vi "Get Input.vi"(8 "error in (no error)":errorcluster, 10 "DIO_CFG":refnum<class "DIO-Configuration.lvclass">, 11 "UI Template in":refnum<class "DIO_Panel.lvclass">) -> (0 "error out":errorcluster, 2 "Input":bool, 3 "UI Template out":refnum<class "DIO_Panel.lvclass">)   [LabVIEW 2021, in "Simulator-Channel.lvlib" / "DIO_Panel.lvlib" / "DIO_Panel.lvclass"]
uses:
  DIO_Panel.lvclass
  Dependencies/DIO-Channel.lvlibp/Channels/DIO-Channel/DIO-Configuration_class/DIO-Configuration.lvclass
  C:/Users/averna/Documents/LV Gym DEMO/Factory Pattern/Channels/Dependencies/Channel.lvlibp/Channel/Configuration_class/Configuration.lvclass
  DIO_Panel.lvclass/DIO_Panel.ctl
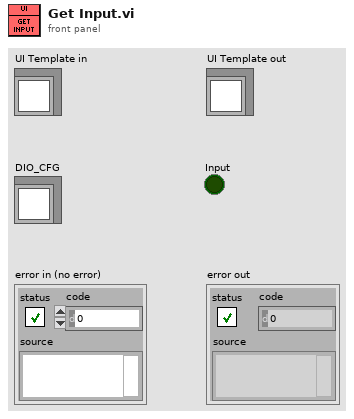
[diagram p1: front panel]
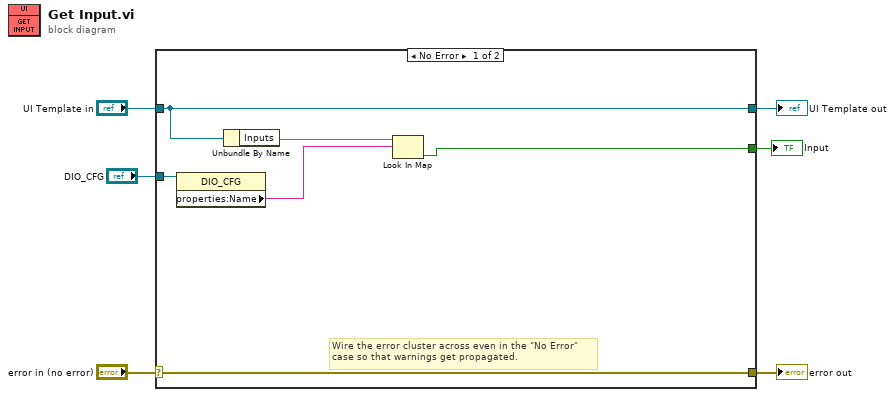
[diagram p0: block diagram]
diagram:
  n1 = case shown="No Error" "error in (no error)" {
    selector: "error in (no error)" -> [w12 w14]
    tunnel: [w12 w14] -> w5
    tunnel: [w11 w13] -> w3
    tunnel: "UI Template in" -> [w11 w13]
    tunnel: "DIO_CFG" -> [w9 _]
    tunnel: [w7 _] -> w1
    frame No Error {
      # "Wire the error cluster across even in the \"No Error\"\ncase so that warnings get propagated."
      n2 = property class="DIO_CFG"(reference=w9) -> ("properties:Name"=w8:string)  [unwired: 1 in, 2 out]
      n3 = Unbundle By Name(w11) -> ("Inputs"=w10:map{string, bool})
      n4 = Look In Map(map=w10, key=w8) -> (value=w7:bool)  [unwired: 1 in, 1 out]
    }
    frame Error {
    }
  }
  "error out" <- w5
  "UI Template out" <- w3
  "Input" <- w1
